vi "PicoScope4000aPowerSource.vi"(6 "USB 3.0 on non-USB 3.0 port control":bool, 7 "Mode":u16(ring) items=["Dialog On Error", "no dialog - CloseUnit and Stop", "no dialog - Continue", "no dialog - Stop"], 8 "USB powered control":bool, 9 "handle in":i16, 10 "PICO STATUS IN":u32 format="%#.0f", 11 "error in (no error)":errorcluster) -> (0 "USB powered":bool, 1 "handle out":i16, 2 "PICO STATUS OUT":u32, 3 "error out":errorcluster, 4 "USB 3.0 on non-USB 3.0 port":bool)   [LabVIEW 2009]
uses:
  ps4000A.dll
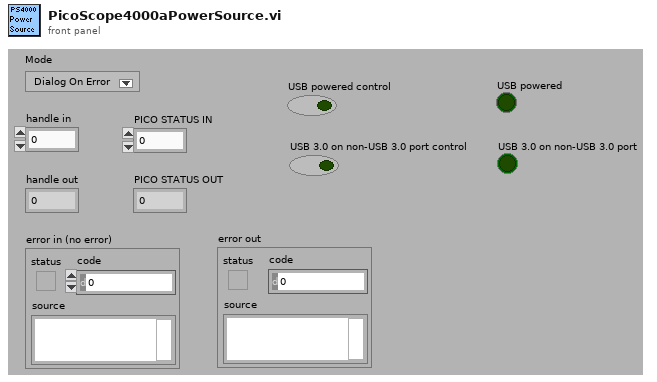
[diagram p1: front panel]
types:
  T1 = cluster{"status":bool, "code":u32, "source":string}
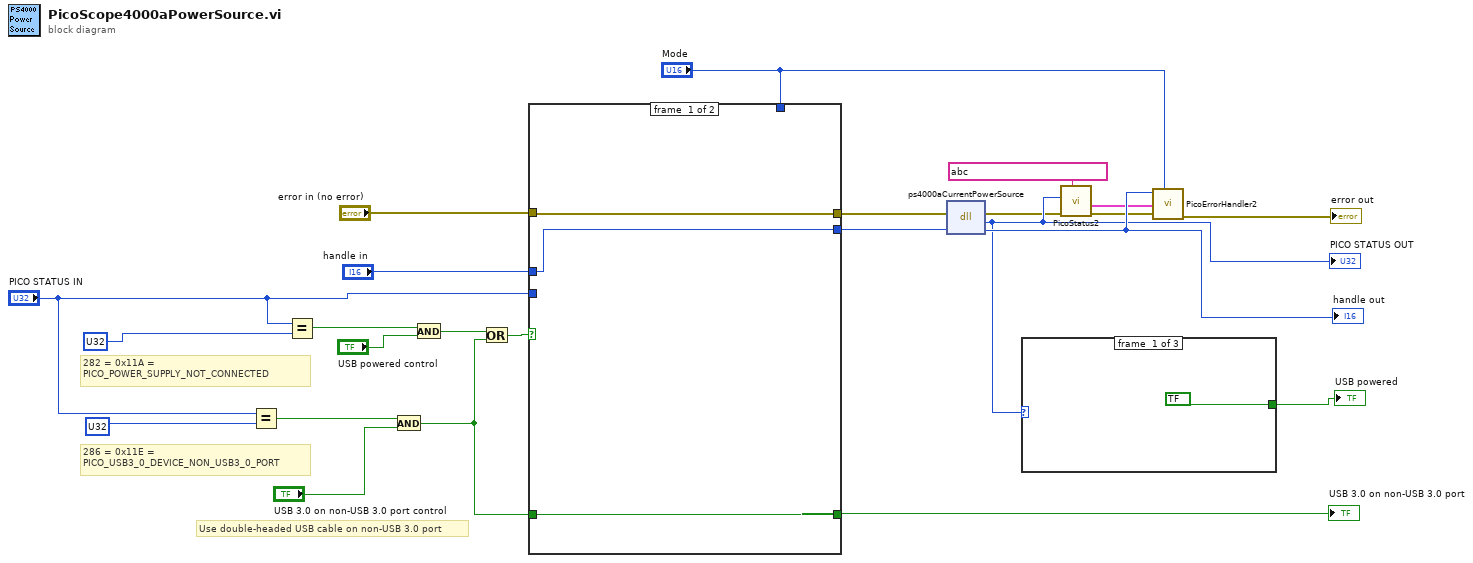
[diagram p0: block diagram]
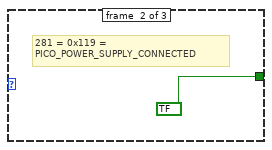
[diagram p2: hidden frame]
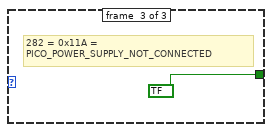
[diagram p3: hidden frame]
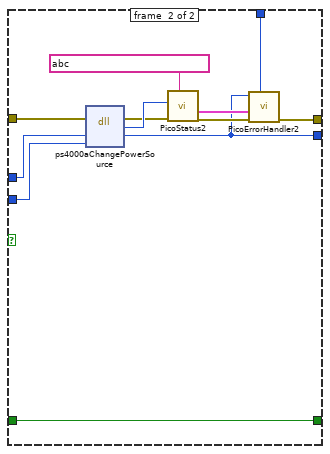
[diagram p4: hidden frame]
diagram:
  # "Use double-headed USB cable on non-USB 3.0 port"
  # "282 = 0x11A = \nPICO_POWER_SUPPLY_NOT_CONNECTED"
  # "286 = 0x11E = \nPICO_USB3_0_DEVICE_NON_USB3_0_PORT"
  n1 = Equal?(x="PICO STATUS IN", y=u32 ?) -> (x = y?=w21:bool)
  n2 = Equal?(x="PICO STATUS IN", y=u32 ?) -> (x = y?=w17:bool)
  n3 = And(x=w21, y="USB 3.0 on non-USB 3.0 port control") -> (x .and. y?=w13:bool)
  n4 = And(x=w17, y="USB powered control") -> (x .and. y?=w15:bool)
  n5 = Or(x=w15, y=w13) -> (x .or. y?=w14:bool)
  n6 = case shown="True" w14 {
    tunnel: "PICO STATUS IN" -> [_ w38]
    tunnel: "error in (no error)" -> [w25 w39]
    tunnel: "handle in" -> [w27 w37]
    tunnel: [w27 w28] -> w12
    tunnel: w13 -> [w26 w36]
    tunnel: [w26 w36] -> w11
    tunnel: "Mode" -> [_ w32]
    tunnel: [w25 w31] -> w1
    frame #0 {
    }
    frame #1 {
      n7 = dll-call lib="ps4000A.dll" fn="ps4000aChangePowerSource"(error in=w39, "handle"=w37, "powerSource"=w38) -> (error out=w33:errorcluster, "PICO_STATUS"=w34:u32, "handle"=w28:i16)  [unwired: 3 in, 1 out]
      n8 = call "PicoStatus2.vi"("PICO source"=string ? ("source"), "Error in"=w33, "PICO STATUS"=w34) -> ("error out"=w30:errorcluster, "PICO_STATUS out"=w29:T1)  [unwired: 5 in]
      n9 = call "PicoErrorHandler2.vi"("Mode"=w32, "error in (no error)"=w30, "PICO_STATUS in"=w29, "handle In"=w28) -> ("error out"=w31:errorcluster)  [unwired: 7 in]
    }
  }
  "USB 3.0 on non-USB 3.0 port" <- w11
  n10 = dll-call lib="ps4000A.dll" fn="ps4000aCurrentPowerSource"(error in=w1, "handle"=w12) -> (error out=w3:errorcluster, "PICO_STATUS"=w4:u32, "handle"=w9:i16)  [unwired: 2 in, 1 out]
  "PICO STATUS OUT" <- w4
  "handle out" <- w9
  n11 = case shown="282" w4 {
    tunnel: [bool ? bool ? bool ?] -> w10
    frame #0 {
    }
    frame #1 {
      # "281 = 0x119 = \nPICO_POWER_SUPPLY_CONNECTED"
    }
    frame #2 {
      # "282 = 0x11A = \nPICO_POWER_SUPPLY_NOT_CONNECTED"
    }
  }
  "USB powered" <- w10
  n12 = call "PicoStatus2.vi"("PICO source"=string ? ("source"), "Error in"=w3, "PICO STATUS"=w4) -> ("error out"=w7:errorcluster, "PICO_STATUS out"=w6:T1)  [unwired: 5 in]
  n13 = call "PicoErrorHandler2.vi"("Mode"="Mode", "error in (no error)"=w7, "PICO_STATUS in"=w6, "handle In"=w9) -> ("error out"=→"error out":errorcluster)  [unwired: 7 in]
